vi "FuncVI-Pi.vi"(5 "InstanceRef":T2, 9 "arg list":T1[](array[typedef]) {"num" format="%.2f"}) -> (0 "error out":bool, 3 "result":T1 {"num" format="%.2f"})   [LabVIEW 2021]
doc: "::: CalcExpress Toolkit :::\nCopyright (c) 2000-2026 Konstantin Shifershteyn. All rights reserved."
uses:
  cetypes.llb/CalcExpress Function Argument Info.ctl
  cetypes.llb/CalcExpress Instance RefNum.ctl
panel:
  in  "max arg num":i32=1
  in  "min arg num":i32
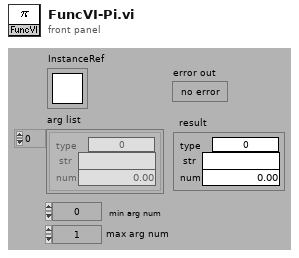
[diagram p1: front panel]
types:
  T1 = typedef "CalcExpress Function Argument Info.ctl" = cluster{"type":u32, "str":string, "num":dbl}
  T2 = typedef "CalcExpress Instance RefNum.ctl" = refnum<k1>
  T3 = enum32{"String", "DBL Number", "identifier", "1D Array of DBL", "2D Array of DBL", "CDB Number", "1D Array of CDB", "2D Array of CDB", "1D Array of String", "2D Array of String", "Unknown data type"}
  T4 = cluster{"data type":enum32{"String", "DBL Number", "identifier", "1D Array of DBL", "2D Array of DBL", "CDB Number", "1D Array of CDB", "2D Array of CDB", "1D Array of String", "2D Array of String", "Unknown data type"}, string, dbl}
  T5 = enum16{"DBL scalar", "CDB scalar", "DBL array", "CDB array", "ERROR"}
  T6 = typedef "CalcExpress Data Type.ctl" = enum32{"String", "DBL Number", "identifier", "1D Array of DBL", "2D Array of DBL", "CDB Number", "1D Array of CDB", "2D Array of CDB", "1D Array of String", "2D Array of String", "Unknown data type"}
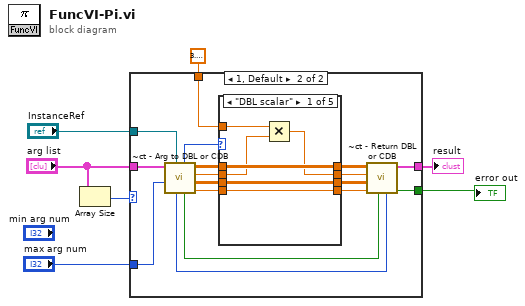
[diagram p0: block diagram]
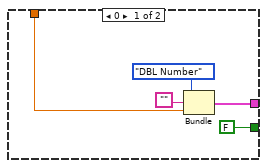
[diagram p2: hidden frame]
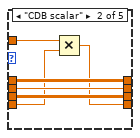
[diagram p3: hidden frame]
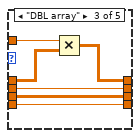
[diagram p4: hidden frame]
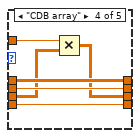
[diagram p5: hidden frame]
diagram:
  n1 = Array Size(array="arg list") -> (size(s)=w4:i32)
  n2 = case shown="1, Default" w4 {
    tunnel: [FALSE ("error out") w29] -> w7
    tunnel: [w9 w28] -> w6
    tunnel: "arg list" -> [_ w27]
    tunnel: "InstanceRef" -> [_ w26]
    tunnel: 3.141592653589793 -> [w8 w14]
    tunnel: "max arg num" -> [_ w13]
    frame 0 {
      n3 = Bundle("data type"=T3."DBL Number", "", w8) -> (w9:T4)  [unwired: 1 in]
    }
    frame 1, Default {
      n4 = call "~ct - Arg to DBL or CDB.vi"("InstanceRef"=w26, "max args"=w13, "args list"=w27) -> ("CDB"=w22:cdb, "2D CDB"=w23:cdb[][], "DBL"=w21:dbl, "2D DBL"=w20:dbl[][], "error out"=w25:bool, "category"=w15:T5, "arg type"=w24:T6)  [unwired: 2 in]
      n5 = case shown="\"DBL scalar\"" w15 {
        tunnel: w23 -> [w34 w40 w47 w49 w54]
        tunnel: w22 -> [w33 w37 w46 w52 w55]
        tunnel: w21 -> [w32 w38 w44 w50 w56]
        tunnel: w20 -> [w35 w41 w43 w53 w57]
        tunnel: [w35 w41 w42 w53 w57] -> w19
        tunnel: [w31 w38 w44 w50 w56] -> w18
        tunnel: [w34 w40 w47 w48 w54] -> w17
        tunnel: [w33 w36 w46 w52 w55] -> w16
        tunnel: w14 -> [w30 w39 w45 w51 _]
        frame "DBL scalar" {
          n6 = Multiply(x=w30, y=w32) -> (x*y=w31:dbl)
        }
        frame "CDB scalar" {
          n7 = Multiply(x=w39, y=w37) -> (x*y=w36:cdb)
        }
        frame "DBL array" {
          n8 = Multiply(x=w45, y=w43) -> (x*y=w42:dbl[][])
        }
        frame "CDB array" {
          n9 = Multiply(x=w51, y=w49) -> (x*y=w48:cdb[][])
        }
        frame "ERROR" {
        }
      }
      n10 = call "~ct - Return DBL or CDB.vi"("type"=w24, "error in"=w25, "CDB"=w16, "2D CDB"=w17, "DBL"=w18, "2D DBL"=w19) -> ("error out"=w29:bool, "result"=w28:T1)  [unwired: 4 in]
    }
  }
  "error out" <- w7
  "result" <- w6
